vi "~ct - Return DBL or CDB.vi"(4 "type":T1, 6 "error in":bool, 8 "CDB":cdb format="%.2f", 9 "2D CDB":cdb[][](array[numeric]) format="%.2f", 10 "DBL":dbl format="%.2f", 11 "2D DBL":dbl[][](array[numeric]) format="%.2f") -> (0 "error out":bool, 3 "result":T2)   [LabVIEW 2021]
doc: "::: CalcExpress Toolkit :::\nCopyright (c) 2000-2026 Konstantin Shifershteyn. All rights reserved."
uses:
  cetypes.llb/CalcExpress Function Argument Info.ctl
  cetypes.llb/CalcExpress Data Type.ctl
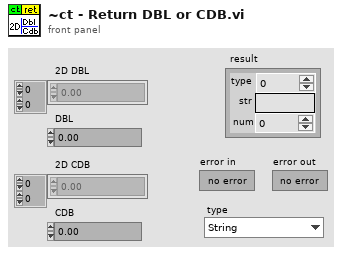
[diagram p1: front panel]
types:
  T1 = typedef "CalcExpress Data Type.ctl" = enum32{"String", "DBL Number", "identifier", "1D Array of DBL", "2D Array of DBL", "CDB Number", "1D Array of CDB", "2D Array of CDB", "1D Array of String", "2D Array of String", "Unknown data type"}
  T2 = typedef "CalcExpress Function Argument Info.ctl" = cluster{"type":u32, "str":string, "num":dbl}
  T3 = enum32{"String", "DBL Number", "identifier", "1D Array of DBL", "2D Array of DBL", "CDB Number", "1D Array of CDB", "2D Array of CDB", "1D Array of String", "2D Array of String", "Unknown data type"}
  T4 = cluster{"type":T1, "data string":string, "DBL":dbl}
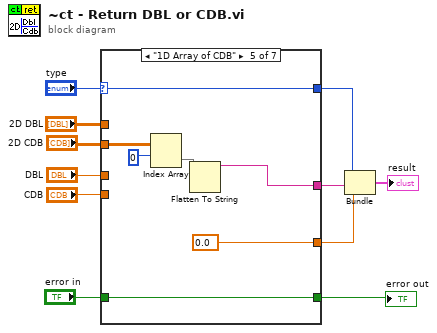
[diagram p0: block diagram]
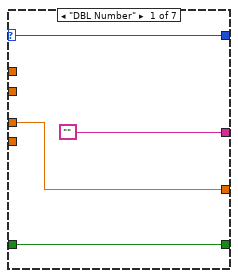
[diagram p2: hidden frame]
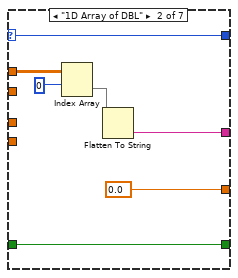
[diagram p3: hidden frame]
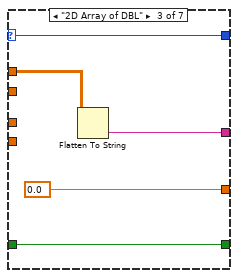
[diagram p4: hidden frame]
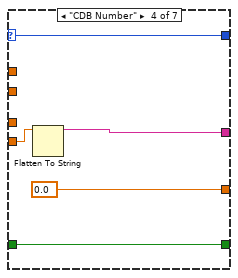
[diagram p5: hidden frame]
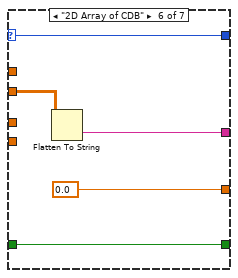
[diagram p6: hidden frame]
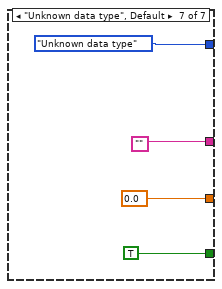
[diagram p7: hidden frame]
diagram:
  n1 = case shown="\"1D Array of CDB\"" "type" {
    selector: "type" -> [w13 w18 w24 w29 w35 w41 _]
    tunnel: ["" w22 w27 w30 w39 w44 ""] -> w8
    tunnel: "2D CDB" -> [_ _ _ _ w36 w43 _]
    tunnel: [w14 0.0 0.0 0.0 0.0 0.0 0.0] -> w7
    tunnel: "CDB" -> [_ _ _ w31 _ _ _]
    tunnel: "DBL" -> [w14 _ _ _ _ _ _]
    tunnel: "2D DBL" -> [_ w20 w25 _ _ _ _]
    tunnel: [w13 w18 w24 w29 w35 w41 T3."Unknown data type" ("left type")] -> w1
    tunnel: "error in" -> [w12 w17 w23 w28 w34 w40 _]
    tunnel: [w12 w17 w23 w28 w34 w40 TRUE ("error in")] -> w2
    frame "DBL Number" {
    }
    frame "1D Array of DBL" {
      n2 = Index Array(array=w20, index (row)=0) -> (element=w19:dbl[])  [unwired: 1 in]
      n3 = Flatten To String(anything=w19) -> (data string=w22:string)  [unwired: 3 in, 2 out]
    }
    frame "2D Array of DBL" {
      n4 = Flatten To String(anything=w25) -> (data string=w27:string)  [unwired: 3 in, 2 out]
    }
    frame "CDB Number" {
      n5 = Flatten To String(anything=w31) -> (data string=w30:string)  [unwired: 3 in, 2 out]
    }
    frame "1D Array of CDB" {
      n6 = Index Array(array=w36, index (row)=0) -> (element=w38:cdb[])  [unwired: 1 in]
      n7 = Flatten To String(anything=w38) -> (data string=w39:string)  [unwired: 3 in, 2 out]
    }
    frame "2D Array of CDB" {
      n8 = Flatten To String(anything=w43) -> (data string=w44:string)  [unwired: 3 in, 2 out]
    }
    frame "Unknown data type", Default {
    }
  }
  "error out" <- w2
  n9 = Bundle("type"=w1, "data string"=w8, "DBL"=w7) -> (→"result":T4)  [unwired: 1 in]
